vi "RDC-coax-calculate_from_meas.vi"(7 "dielectric":T1, 11 "measurement":T3) -> (1 "lenght array":dbl[](graph), 2 "lenght [m]":dbl format="%#_6p", 3 "tau":dbl format="%#_6p")   [LabVIEW 2020, in "RDC-Reflection_Data_Computation.lvlib"]
doc: "Calculates the coax length (in m) and the delay tau from the phase of a measured Common Format cluster and the selected coax dielectric. Also returns the length per frequency."
uses:
  RDC-Reflection_Data_Computation.lvlib
  Reflector/RFH-common_data_format.ctl
  RDC-dielectric_types.ctl
  <vilib>/Analysis/6fits.llb/Curve Fitting Criteria.ctl
  30b2abce-0734-4a3c-a09c-f206fb615947.vi
  <vilib>/Analysis/NI_AALPro.lvlib
  Reflector/RFH-Reflection_File_Handler.lvlib
panel:
  out "2phi":dbl[](array[numeric])
  out "Phi":dbl[](array[numeric])
  out "k":dbl[](array[numeric])
  in  "index":i32
  out "Tau":cluster{"Frequency":dbl[], dbl[]}(graph)
  out "AVG":dbl
  out "fitting":T2(graph)
  out "unwrapping":T2(graph)
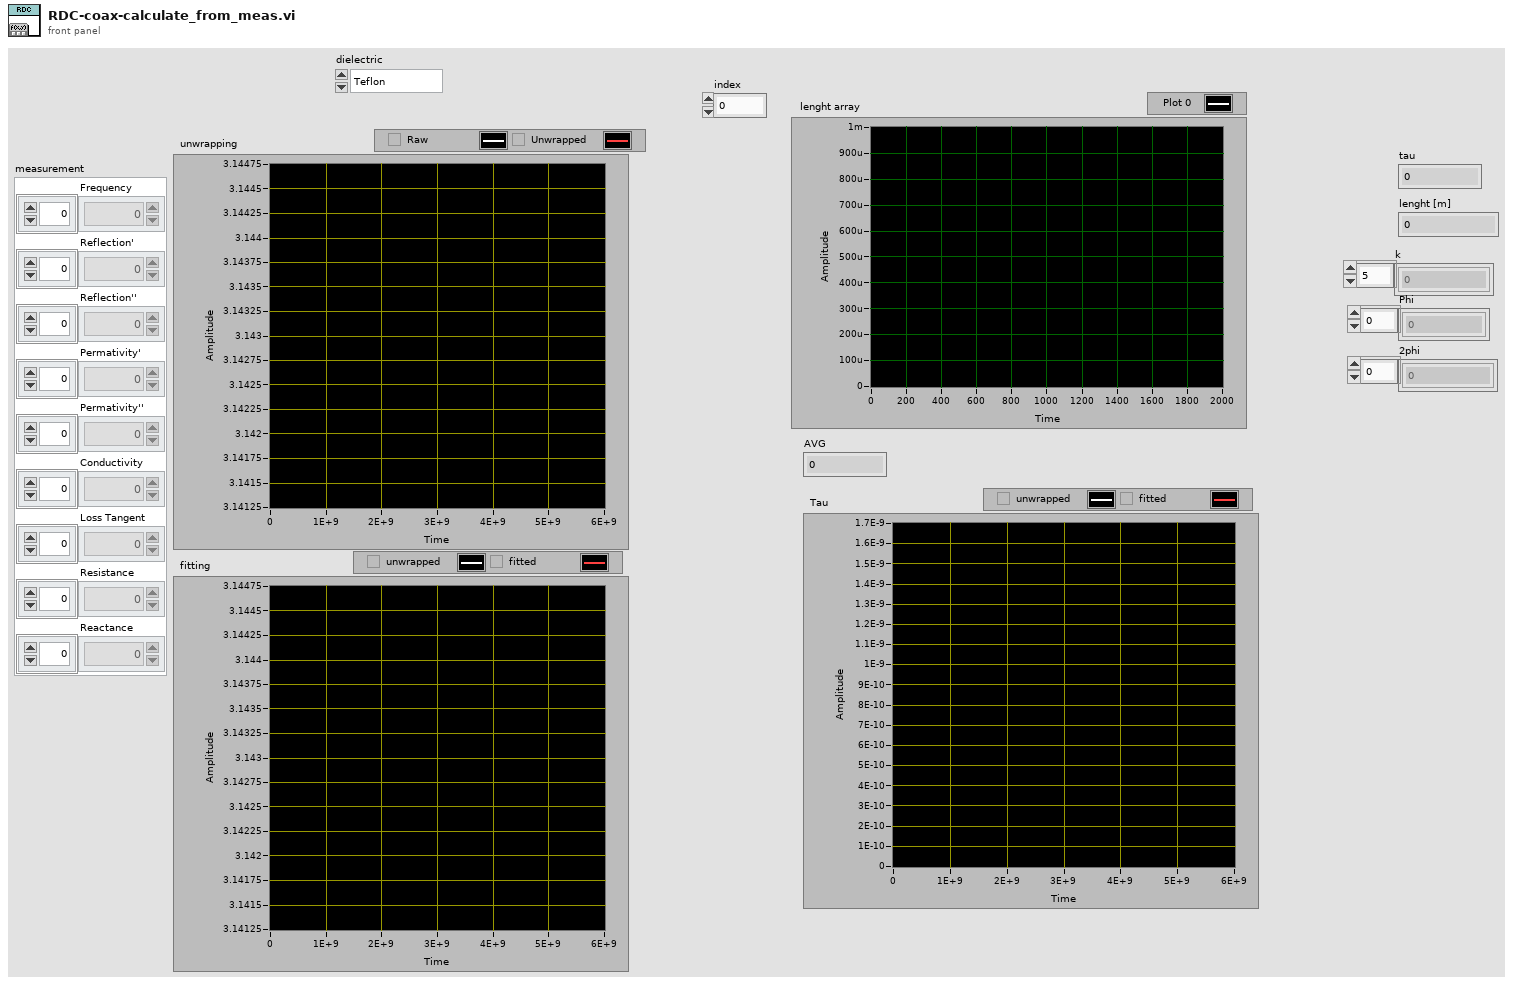
[diagram p1: front panel]
types:
  T1 = typedef "RDC-Reflection_Data_Computation.lvlib/RDC-dielectric_types.ctl" = enum16{"Teflon", "Eccostock 0005"}
  T2 = cluster{"Frequency":dbl[], "Reflection''":dbl[]}[]
  T3 = typedef "RFH-Reflection_File_Handler.lvlib/RFH-common_data_format.ctl" = cluster{"Frequency":dbl[], "Reflection'":dbl[], "Reflection''":dbl[], "Permativity'":dbl[], "Permativity''":dbl[], "Conductivity":dbl[], "Loss Tangent":dbl[], "Resistance":dbl[], "Reactance":dbl[]}
  T4 = cluster{"Frequency":dbl[], "Unwrapped Phase":dbl[]}
  T5 = cluster{"Frequency":dbl[], "Unwrapped Phase":dbl[]}[]
  T6 = typedef "NI_AALPro.lvlib/Curve Fitting Criteria.ctl" = u16
  T7 = cluster{"Frequency":dbl[], "Best Linear Fit":dbl[]}
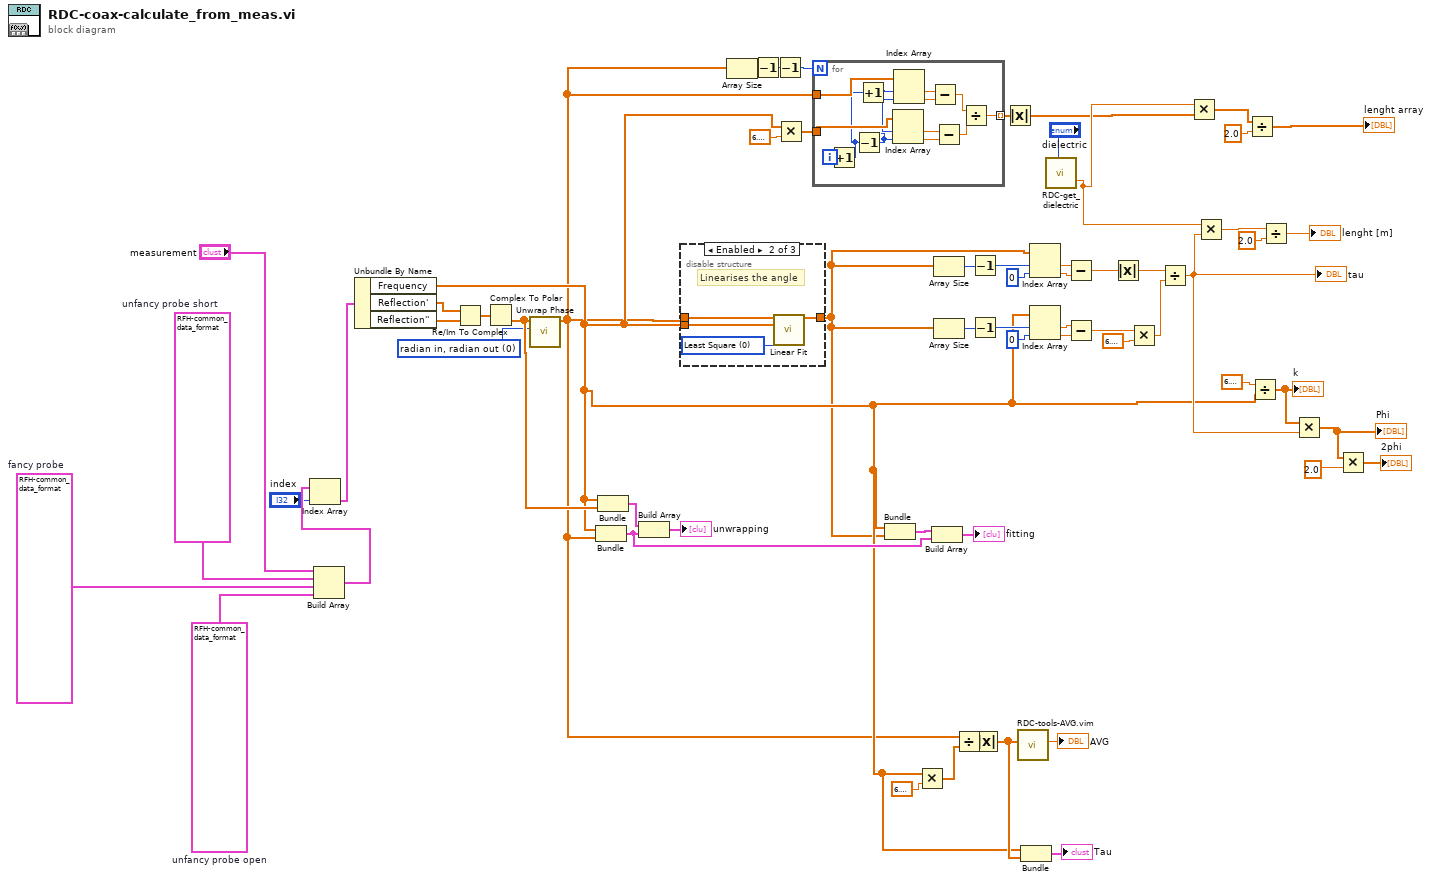
[diagram p0: block diagram]
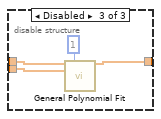
[diagram p3: hidden frame]
diagram:
  w26 = T3 {"Frequency"=array[2001 elements], "Reflection'"=array[2001 elements], "Reflection''"=array[2001 elements], "Permativity'"=array[2001 elements], "Permativity''"=array[2001 elements], "Conductivity"=array[2001 elements], "Loss Tangent"=array[2001 elements], "Resistance"=array[2001 elements], "Reactance"=array[2001 elements]}  # unfancy probe open
  w27 = T3 {"Frequency"=array[2001 elements], "Reflection'"=array[2001 elements], "Reflection''"=array[2001 elements], "Permativity'"=array[2001 elements], "Permativity''"=array[2001 elements], "Conductivity"=array[2001 elements], "Loss Tangent"=array[2001 elements], "Resistance"=[], "Reactance"=[]}  # fancy probe
  w28 = T3 {"Frequency"=array[2001 elements], "Reflection'"=array[2001 elements], "Reflection''"=array[2001 elements], "Permativity'"=array[2001 elements], "Permativity''"=array[2001 elements], "Conductivity"=array[2001 elements], "Loss Tangent"=array[2001 elements], "Resistance"=array[2001 elements], "Reactance"=array[2001 elements]}  # unfancy probe short
  w56 = 0 items=["radian in, radian out", "radian in, degree out", "degree in, degree out", "degree in, radian out"] ("phase unit")
  n1 = Build Array("measurement", w28, w27, w26) -> (w25:T3[])
  n2 = Index Array(array=w25, index="index") -> (element=w15:T3)
  n3 = Unbundle By Name(w15) -> ("Frequency"=w12:dbl[], "Reflection'"=w59:dbl[], "Reflection''"=w58:dbl[])
  n4 = Re/Im To Complex(1:w58, 2:w59) -> (0:w61:cdb[])
  n5 = Complex To Polar(r * e^(i*theta)=w61) -> (theta=w57:dbl[])  [unwired: 1 out]
  n6 = call <vilib>:"Unwrap Phase.vi"("phase unit"=w56, "Phase"=w57) -> ("Unwrapped Phase"=w8:dbl[])  [unwired: 8 in, 1 out]
  n7 = Bundle("Frequency"=w12, "Unwrapped Phase"=w8) -> (w53:T4)  [unwired: 1 in]
  n8 = Bundle("Frequency"=w12, w57) -> (w60:cluster{"Frequency":dbl[], dbl[]})  [unwired: 1 in]
  n9 = Build Array(w60, w53) -> (→"unwrapping":T5)
  n10 = disable-structure shown="Enabled" {
    disable-tunnel: w12 -> [_ w66 w69]
    disable-tunnel: [w63 w65 w68] -> w11
    disable-tunnel: w8 -> [w63 w64 w70]
    frame Disabled {
    }
    frame Enabled {
      w67 = T6 0 items=["Least Square", "Least Absolute Residual", "Bisquare"] ("method")
      # "Linearises the angle"
      n11 = call <vilib>:"Linear Fit.vi"("Y"=w64, "X"=w66, "method"=w67) -> ("Best Linear Fit"=w65:dbl[])  [unwired: 8 in, 4 out]
    }
    frame Disabled {
      n12 = call <vilib>:"General Polynomial Fit.vi"("Y"=w70, "polynomial order"=1, "X"=w69) -> ("Best Polynomial Fit"=w68:dbl[])  [unwired: 9 in, 3 out]
    }
  }
  n13 = Array Size(array=w8) -> (size(s)=w10:i32)
  n14 = Decrement(x=w10) -> (x-1=w9:i32)
  n15 = Decrement(x=w9) -> (x-1=w6:i32)
  n16 = Multiply(x=w12, y=6.283185307179586) -> (x*y=w7:dbl[])
  n17 = for {
    N: w6 -> [_]
    tunnel: w8 -> [w84]
    tunnel: w7 -> [w82]
    tunnel: [w72] -> w5 mode=indexing
    i -> [w78]
    n18 = Increment(x=w78) -> (x+1=w76:i32)
    n19 = Decrement(x=w76) -> (x-1=w75:i32)
    n20 = Increment(x=w76) -> (x+1=w77:i32)
    n21 = Index Array(array=w82, index #1=w77, index #2=w75) -> (element #1=w80:dbl, element #2=w81:dbl)
    n22 = Index Array(array=w84, index #1=w77, index #2=w75) -> (element #1=w79:dbl, element #2=w83:dbl)
    n23 = Subtract(x=w79, y=w83) -> (x-y=w74:dbl)
    n24 = Subtract(x=w80, y=w81) -> (x-y=w73:dbl)
    n25 = Divide(x=w74, y=w73) -> (x/y=w72:dbl)
  }
  n26 = Bundle("Frequency"=w12, "Best Linear Fit"=w11) -> (w55:T7)  [unwired: 1 in]
  n27 = Multiply(x=w12, y=6.283185307179586) -> (x*y=w36:dbl[])
  n28 = Build Array(w55, w53) -> (→"fitting":T5)
  n29 = Array Size(array=w11) -> (size(s)=w50:i32)
  n30 = Array Size(array=w11) -> (size(s)=w44:i32)
  n31 = Divide(x=w8, y=w36) -> (x/y=w34:dbl[])
  n32 = Decrement(x=w50) -> (x-1=w47:i32)
  n33 = Decrement(x=w44) -> (x-1=w45:i32)
  n34 = Absolute Value(x=w34) -> (abs(x)=w23:dbl[])
  n35 = Absolute Value(x=w5) -> (abs(x)=w1:dbl[])
  n36 = call "RDC-tools-AVG.vim"("Data Array"=w23) -> ("AVG"=→"AVG":dbl)  [unwired: 10 in]
  n37 = Bundle("Frequency"=w12, w23) -> (→"Tau":cluster{"Frequency":dbl[], dbl[]})  [unwired: 1 in]
  n38 = Index Array(array=w11, index #1=w47, index #2=0 ("index")) -> (element #1=w52:dbl, element #2=w46:dbl)
  n39 = Index Array(array=w12, index #1=w45, index #2=0 ("index")) -> (element #1=w41:dbl, element #2=w42:dbl)
  n40 = call "RDC-get_dielectric.vi"("dielectric"="dielectric") -> ("Vp"=w16:dbl)  [unwired: 13 in, 5 out]
  n41 = Subtract(x=w52, y=w46) -> (x-y=w49:dbl)
  n42 = Subtract(x=w41, y=w42) -> (x-y=w40:dbl)
  n43 = Absolute Value(x=w49) -> (abs(x)=w48:dbl)
  n44 = Multiply(x=w40, y=6.283185307179586) -> (x*y=w38:dbl)
  n45 = Divide(x=w48, y=w38) -> (x/y=w17:dbl)
  "tau" <- w17
  n46 = Multiply(x=w16, y=w1) -> (x*y=w3:dbl[])
  n47 = Multiply(x=w16, y=w17) -> (x*y=w31:dbl)
  n48 = Divide(x=w3, y=2.0) -> (x/y=→"lenght array":dbl[])
  n49 = Divide(x=6.283185307179586, y=w12) -> (x/y=w21:dbl[])
  "k" <- w21
  n50 = Divide(x=w31, y=2.0) -> (x/y=→"lenght [m]":dbl)
  n51 = Multiply(x=w21, y=w17) -> (x*y=w19:dbl[])
  "Phi" <- w19
  n52 = Multiply(x=w19, y=2.0) -> (x*y=→"2phi":dbl[])
